vi "CP Probability Graph.vi"(11 "CP Probability":dbl[][](array[numeric])) -> (3 "CP Graph Profile":cluster{i32[], dbl[]}[](graph))   [LabVIEW 2018]
panel:
  out "配列":cluster{i32[], dbl[]}[](array[cluster])
  out "サイズ":i32[](array[numeric])
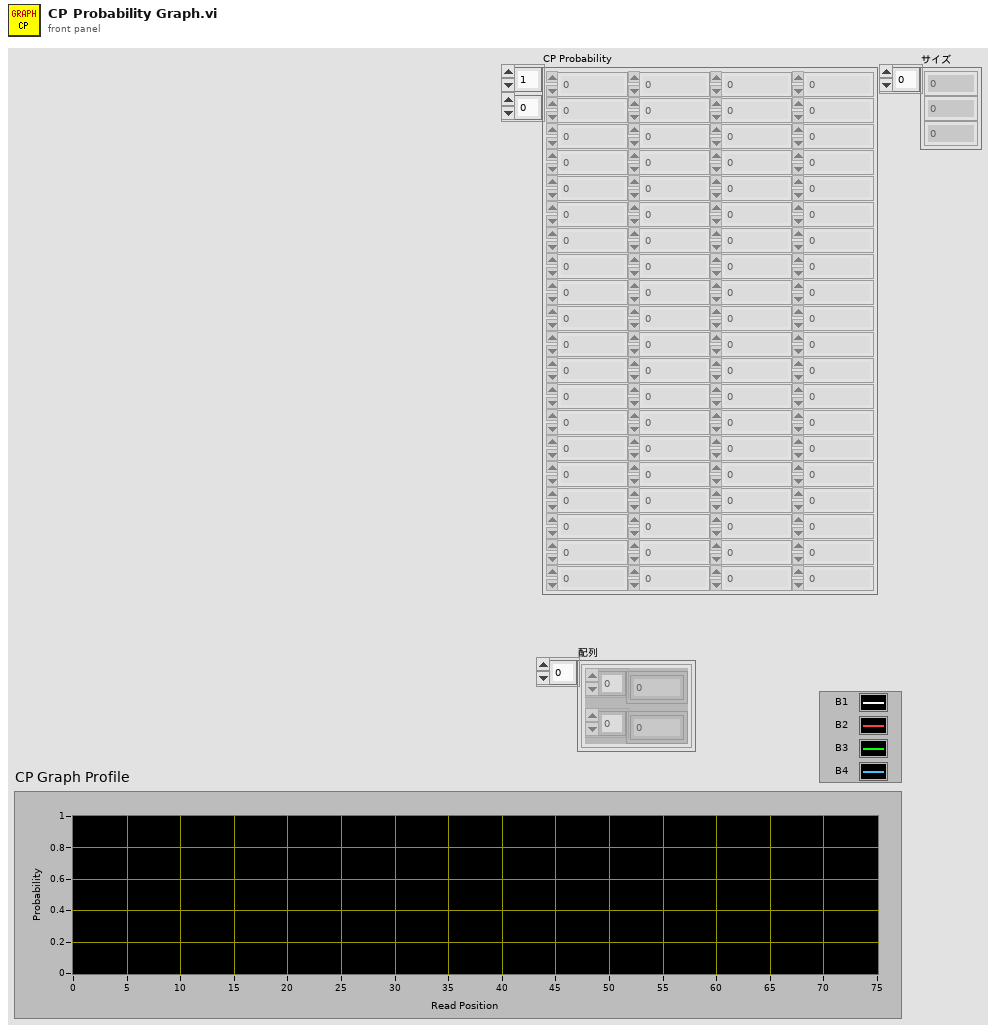
[diagram p1: front panel]
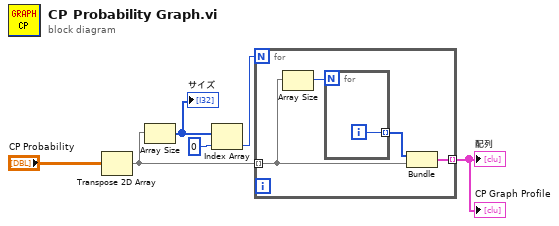
[diagram p0: block diagram]
diagram:
  n1 = Transpose 2D Array(2D array="CP Probability") -> (transposed array=w3:dbl[][])
  n2 = Array Size(array=w3) -> (size(s)=w5:i32[])
  "サイズ" <- w5
  n3 = Index Array(array=w5, index=0 ("指標")) -> (element=w2:i32)
  n4 = for {
    N: w2 -> [_]
    tunnel: w3 -> [w10] mode=indexing
    tunnel: [w7] -> w1 mode=indexing
    n5 = Array Size(array=w10) -> (size(s)=w9:i32)
    n6 = for {
      N: w9 -> [_]
      tunnel: [w11] -> w8 mode=indexing
      i -> [w11]
    }
    n7 = Bundle(w8, w10) -> (w7:cluster{i32[], dbl[]})  [unwired: 1 in]
  }
  "配列" <- w1
  "CP Graph Profile" <- w1
